vi "Test Config Iface Default I32.vi"(8 "error in (no error)":errorcluster, 11 "Test Case In":refnum<class "Configuration Interface Test.lvclass">) -> (0 "error out":errorcluster, 3 "Test Case Out":refnum<class "Configuration Interface Test.lvclass">)   [LabVIEW 2020, in "Configuration Interface Test.lvclass"]
uses:
  Configuration Interface Test.lvclass
  C:/Program Files (x86)/National Instruments/LabVIEW 2020/vi.lib/Astemes/LUnit/Test Case.lvclass
  source/Framework/Configuration/Configuration.lvclass
  <vilib>/Astemes/LUnit/Test Case.lvclass/Test Case.ctl
  6db1c19f-2705-4a91-b5d4-74aaa2a7e517.vi
  <vilib>/Astemes/LUnit/Palette/Pass.vi
  <vilib>/Astemes/LUnit/Palette/Fail.vi
  <vilib>/Astemes/LUnit/Compare Variants.vi
  <vilib>/Astemes/LUnit/Describe Comparison.vi
  <vilib>/Astemes/LUnit/Set Assertion Type.vi
  <vilib>/Astemes/LUnit/Add test result.vi
  <vilib>/Astemes/LUnit/Variant to string.vi
  <vilib>/Astemes/LUnit/LUnit Record Assertion Result.vi
  <vilib>/Astemes/LUnit/LUnit Aggregate Assertion Results.vi
  <vilib>/Astemes/LUnit/Method Result/LUnit Merge Status.vi
  <vilib>/Astemes/LUnit/LUnit Concatenate result strings.vi
  <vilib>/Utility/Data Type/Get Type Information.vi
  <vilib>/Utility/LVClass/Get LV Class Name.vi
  Configuration Interface Test.lvclass/Configuration Interface Test.ctl
  <vilib>/Astemes/LUnit/Test Case.lvclass
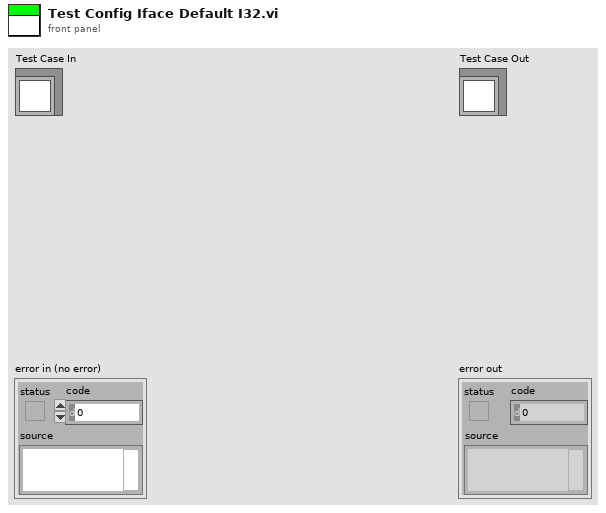
[diagram p1: front panel]
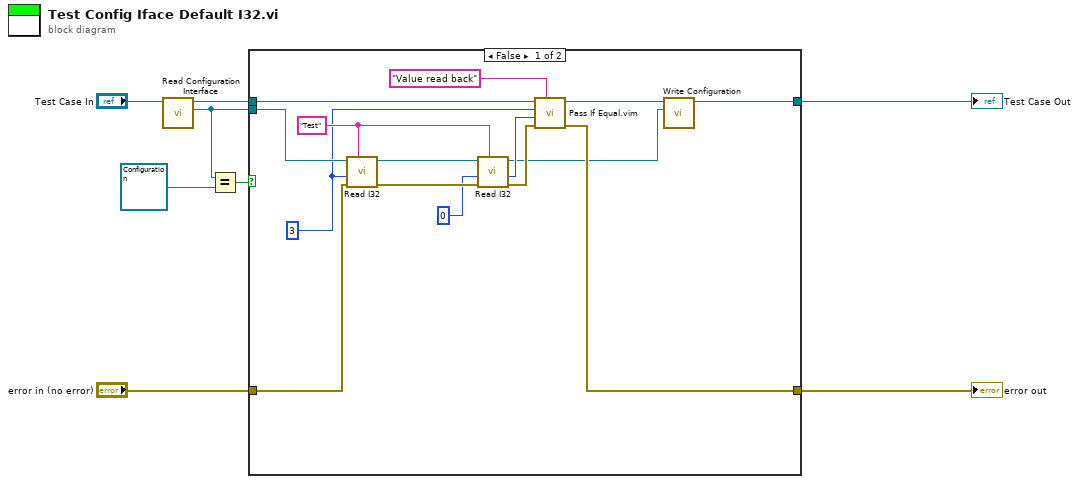
[diagram p0: block diagram]
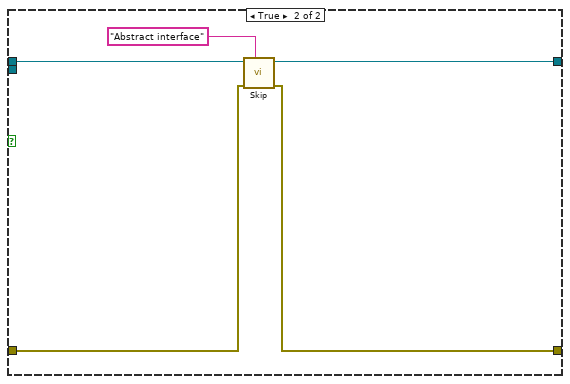
[diagram p2: hidden frame]
diagram:
  n1 = call "Read Configuration Interface.vi"("Configuration Interface Test In"="Test Case In") -> ("Configuration"=w3:refnum<class "Configuration.lvclass">, "Configuration Interface Test Out"=w6:refnum<class "Configuration Interface Test.lvclass">)  [unwired: 9 in]
  n2 = Equal?(x=w3, y=refnum<class "Configuration.lvclass"> refnum ("Configuration")) -> (x = y?=w1:bool)
  n3 = case shown="False" w1 {
    tunnel: [w20 w25] -> w7
    tunnel: w6 -> [w19 w28]
    tunnel: [w10 w27] -> w5
    tunnel: "error in (no error)" -> [w13 w26]
    tunnel: w3 -> [w16 _]
    frame False {
      w12 = 3
      w21 = "Test" ("key")
      n4 = call-dynamic "Read I32.vi"("key"=w21, "error in (no error)"=w13, "default value"=w12, "Configuration In"=w16) -> ("error out"=w22:errorcluster, "Configuration Out"=w23:refnum<class "Configuration.lvclass">)  [unwired: 5 in, 1 out]
      n5 = call-dynamic "Read I32.vi"("key"=w21, "error in (no error)"=w22, "default value"=0, "Configuration In"=w23) -> ("error out"=w17:errorcluster, "value"=w14:i32, "Configuration Out"=w9:refnum<class "Configuration.lvclass">)  [unwired: 5 in]
      n6 = call "Pass If Equal.vim"("Description"="Value read back", "error in (no error)"=w17, "Actual"=w14, "Expected"=w12, "LUnit Test Case In"=w19) -> ("error out"=w20:errorcluster, "LUnit Test Case Out"=w18:refnum<class "Configuration Interface Test.lvclass">)  [unwired: 5 in]
      n7 = call "Write Configuration.vi"("Configuration"=w9, "Configuration Interface Test In"=w18) -> ("Configuration Interface Test Out"=w10:refnum<class "Configuration Interface Test.lvclass">)  [unwired: 8 in, 1 out]
    }
    frame True {
      n8 = call <vilib>:"Skip.vi"("Description"="Abstract interface", "error in (no error)"=w26, "LUnit Test Case In"=w28) -> ("error out"=w25:errorcluster, "LUnit Test Case Out"=w27:refnum<class "Configuration Interface Test.lvclass">)  [unwired: 7 in]
    }
  }
  "error out" <- w7
  "Test Case Out" <- w5
